vi "Query IDN.vi"(8 "error in (no error)":errorcluster, 11 "ETS_EM2090 in":refnum<class "ETS_EM2090.lvclass">) -> (0 "error out":errorcluster, 2 "Connected?":bool, 3 "ETS_EM2090 out":refnum<class "ETS_EM2090.lvclass">)   [LabVIEW 2023, in "Turn Table and Mast.lvlib" / "ETS_EM2090.lvclass"]
uses:
  ETS_EM2090.lvclass
  ETS_EM2090.lvclass/ETS_EM2090.ctl
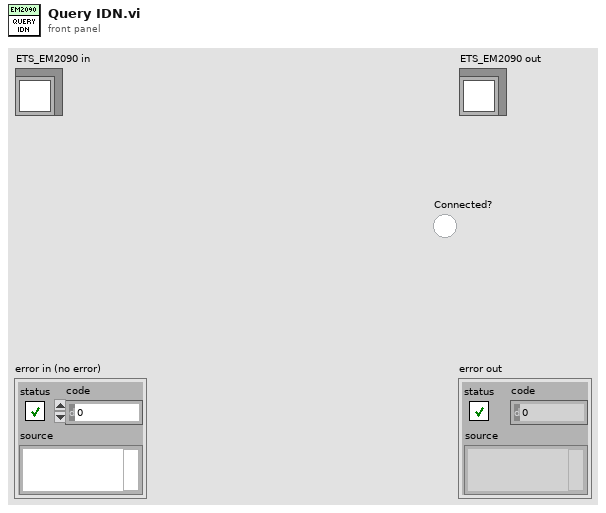
[diagram p1: front panel]
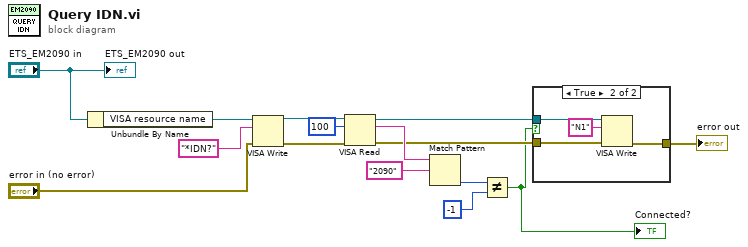
[diagram p0: block diagram]
diagram:
  n1 = Unbundle By Name("ETS_EM2090 in") -> ("VISA resource name"=w1:refnum<visa-resource-name>)
  n2 = VISA Write(VISA resource name=w1, write buffer="*IDN?", error in (no error)="error in (no error)") -> (VISA resource name out=w14:refnum<visa-resource-name>, error out=w13:errorcluster)  [unwired: 1 out]
  n3 = VISA Read(VISA resource name=w14, byte count=u32 100, error in (no error)=w13) -> (VISA resource name out=w5:refnum<visa-resource-name>, read buffer=w11:string, error out=w4:errorcluster)  [unwired: 1 out]
  n4 = Match Pattern(string=w11, regular expression="2090") -> (offset past match=w9:i32)  [unwired: 1 in, 3 out]
  n5 = Not Equal?(x=w9, y=-1) -> (x != y?=w2:bool)
  "Connected?" <- w2
  n6 = case shown="True" w2 {
    tunnel: w5 -> [_ w20]
    tunnel: w4 -> [w16 w19]
    tunnel: [w16 w18] -> w3
    frame False {
    }
    frame True {
      n7 = VISA Write(VISA resource name=w20, write buffer="N1", error in (no error)=w19) -> (error out=w18:errorcluster)  [unwired: 2 out]
    }
  }
  "error out" <- w3
  "ETS_EM2090 out" <- "ETS_EM2090 in"
